vi "PicoScope5000aRunBlock.vi"(7 "Acquisition Settings":T1={"preTriggerSamples"=0, "postTriggerSamples"=1000, "timebase"=2} {"postTriggerSamples" format="%_6p"; "preTriggerSamples" format="%_6p"}, 8 "error in (no error)":errorcluster, 11 "handle in":i16) -> (0 "error out":errorcluster, 3 "handle out":i16, 4 "timeIndisposedMs":dbl, 6 "Total Requested Samples":u64)   [LabVIEW 2010]
doc: "Calls ps5000aRunBlock"
uses:
  ps5000a.dll
  shared/Acquisition Settings.ctl
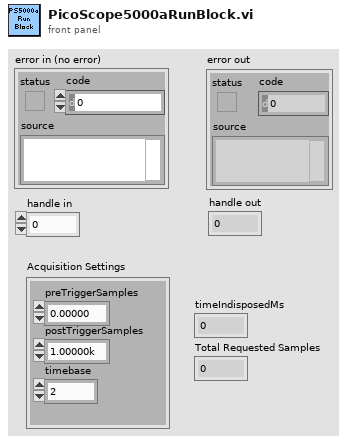
[diagram p1: front panel]
types:
  T1 = typedef "Acquisition Settings.ctl" = cluster{"preTriggerSamples":u64, "postTriggerSamples":u64, "timebase":u32}
  T2 = cluster{"status":bool, "code":u32, "source":string}
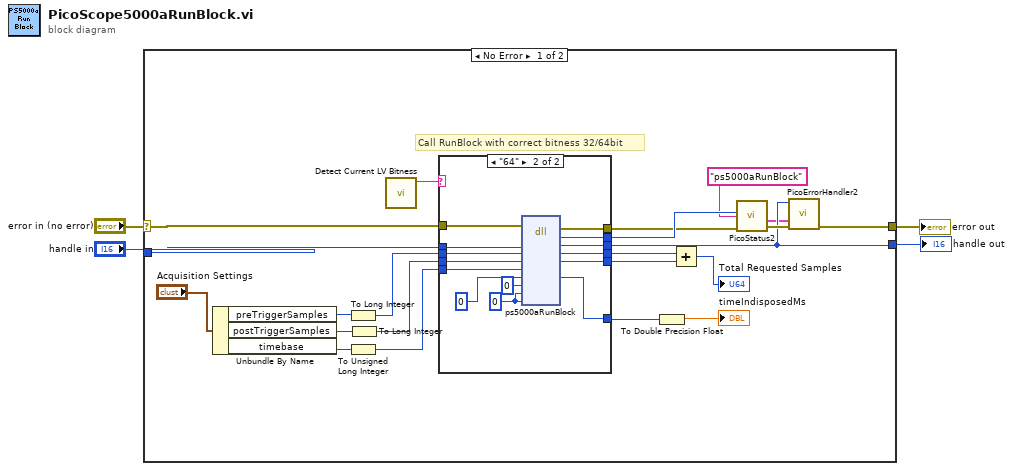
[diagram p0: block diagram]
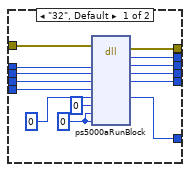
[diagram p2: hidden frame]
diagram:
  n1 = case shown="No Error" "error in (no error)" {
    selector: "error in (no error)" -> [w20 w56]
    tunnel: [w16 w56] -> w2
    tunnel: "handle in" -> [w19 w55]
    tunnel: [w15 w55] -> w3
    frame No Error {
      # "Call RunBlock with correct bitness 32/64bit"
      n2 = Unbundle By Name("Acquisition Settings") -> ("preTriggerSamples"=w13:u64, "postTriggerSamples"=w11:u64, "timebase"=w12:u32)
      n3 = To Long Integer(number=w13) -> (32bit integer=w10:i32)
      n4 = To Unsigned Long Integer(number=w12) -> (unsigned 32bit integer=w8:u32)
      n5 = To Long Integer(number=w11) -> (32bit integer=w9:i32)
      n6 = call "Detect Current LV Bitness.vi"() -> ("bitness"=w17:string)  [unwired: 11 in]
      n7 = case shown="\"64\"" w17 {
        tunnel: [w40 w54] -> w26
        tunnel: [w39 w53] -> w25
        tunnel: [w38 w52] -> w23
        tunnel: [w37 w51] -> w22
        tunnel: w20 -> [w36 w50]
        tunnel: w19 -> [w35 w49]
        tunnel: w10 -> [w33 w47]
        tunnel: w9 -> [w32 w46]
        tunnel: w8 -> [w31 w45]
        tunnel: [w30 w44] -> w15
        tunnel: [w27 w42] -> w6
        frame "32", Default {
          w29 = u32 0 ("pParameter")
          n8 = dll-call lib="ps5000a.dll" fn="ps5000aRunBlock" ("ps3000.dll:_ps3000_open_unit@0")(error in=w36, "handle"=w35, "noOfPreTriggerSamples"=w33, "noOfPostTriggerSamples"=w32, "timebase"=w31, "timeIndisposedMs"=0 ("pParameter"), "segmentIndex"=u32 0, "lpReady"=w29, "pParameter"=w29) -> (error out=w37:errorcluster, "PICO_STATUS"=w38:u32, "handle"=w30:i16, "noOfPreTriggerSamples"=w40:i32, "noOfPostTriggerSamples"=w39:i32, "timeIndisposedMs"=w27:i32)  [unwired: 6 in, 1 out]
        }
        frame "64" {
          w43 = u64 0 ("pParameter")
          n9 = dll-call lib="ps5000a.dll" fn="ps5000aRunBlock" ("ps3000.dll:_ps3000_open_unit@0")(error in=w50, "handle"=w49, "noOfPreTriggerSamples"=w47, "noOfPostTriggerSamples"=w46, "timebase"=w45, "timeIndisposedMs"=0 ("pParameter"), "segmentIndex"=u32 0, "lpReady"=w43, "pParameter"=w43) -> (error out=w51:errorcluster, "PICO_STATUS"=w52:u32, "handle"=w44:i16, "noOfPreTriggerSamples"=w54:i32, "noOfPostTriggerSamples"=w53:i32, "timeIndisposedMs"=w42:i32)  [unwired: 6 in, 1 out]
        }
      }
      n10 = To Double Precision Float(number=w6) -> (double precision float=→"timeIndisposedMs":dbl)
      n11 = Add(x=w26, y=w25) -> (x+y=→"Total Requested Samples":i32)
      n12 = call "PicoStatus2.vi"("PICO source"="ps5000aRunBlock" ("source"), "Error in"=w22, "PICO STATUS"=w23) -> ("error out"=w18:errorcluster, "PICO_STATUS out"=w5:T2)  [unwired: 5 in]
      n13 = call "PicoErrorHandler2.vi"("error in (no error)"=w18, "PICO_STATUS in"=w5, "handle In"=w15) -> ("error out"=w16:errorcluster)  [unwired: 8 in]
    }
    frame Error {
    }
  }
  "error out" <- w2
  "handle out" <- w3
